vi "Build ATM Message.vi"(0 "Message Name":string, 5 "First Name":string, 7 "Last Name":string, 9 "Amount":dbl, 11 "error in":errorcluster) -> (4 "Message":string, 15 "error out":errorcluster)   [LabVIEW 2026, in "ATM.lvlib"]
doc: "Returns the ATM Messages text for a message name, multi-line as in the specification: Welcome, Main Menu (with First Name and Last Name), Verification Failed, Session Terminated, Deposit, Deposit Complete and Withdrawal Complete (with Amount, no decimals when whole), Withdrawal, Withdrawal Failed, Balance Inquiry (the balance on Amount, two decimals). An unknown name returns an empty string. An incoming error passes through."
uses:
  ATM.lvlib
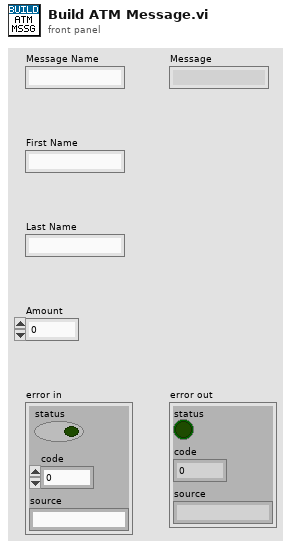
[diagram p1: front panel]
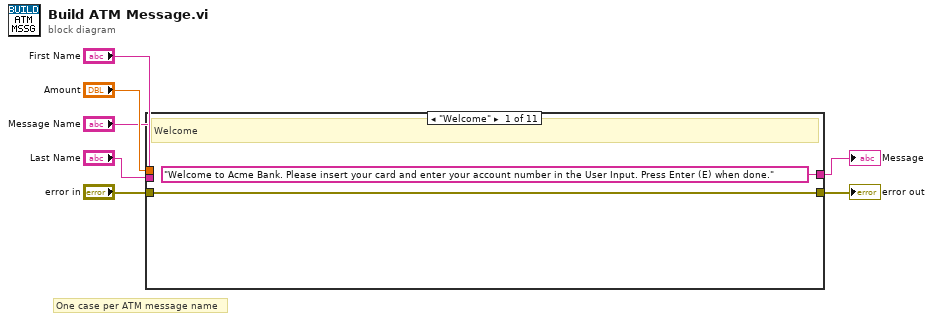
[diagram p0: block diagram]
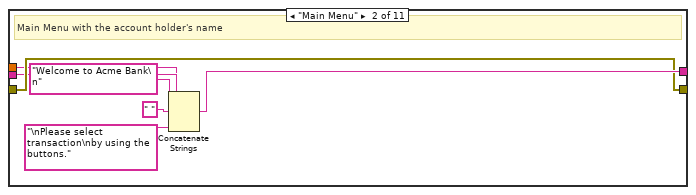
[diagram p2: hidden frame]
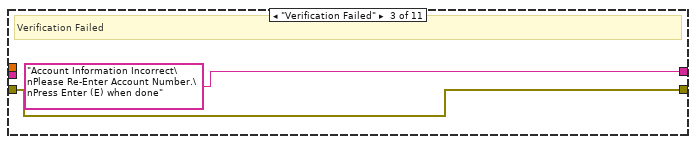
[diagram p3: hidden frame]
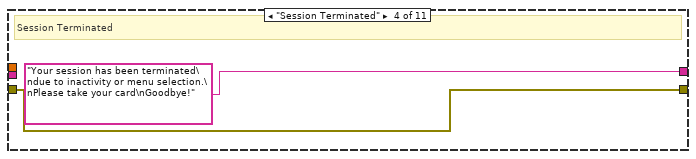
[diagram p4: hidden frame]
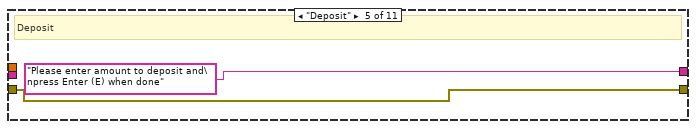
[diagram p5: hidden frame]
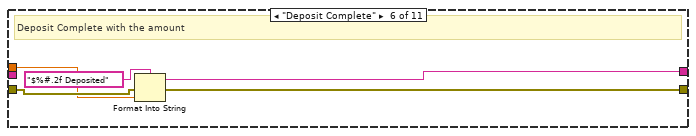
[diagram p6: hidden frame]
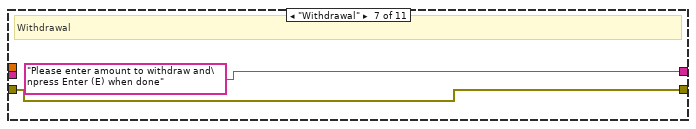
[diagram p7: hidden frame]
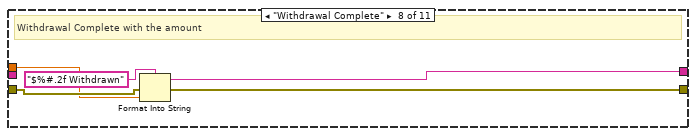
[diagram p8: hidden frame]
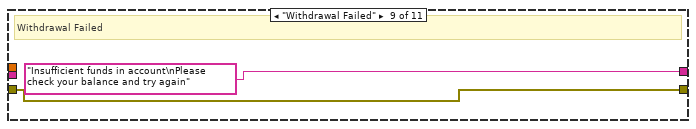
[diagram p9: hidden frame]
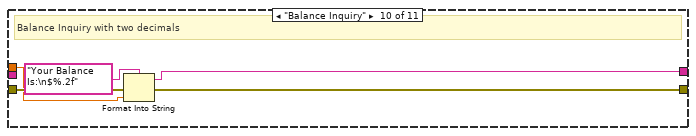
[diagram p10: hidden frame]
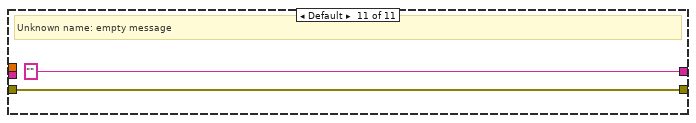
[diagram p11: hidden frame]
diagram:
  # "One case per ATM message name"
  n1 = case shown="\"Welcome\"" "Message Name" {
    tunnel: "First Name" -> [_ w10 _ _ _ _ _ _ _ _ _]
    tunnel: "Last Name" -> [_ w11 _ _ _ _ _ _ _ _ _]
    tunnel: "Amount" -> [_ _ _ _ _ w23 _ w30 _ w37 _]
    tunnel: "error in" -> [w8 w12 w17 w19 w21 w24 w28 w31 w35 w38 w42]
    tunnel: ["Welcome to Acme Bank. Please insert your card and enter your account number in the User Input. Press Enter (E) when done." ("Welcome text") w16 "Account Information Incorrect\nPlease Re-Enter Account Number.\nPress Enter (E) when done" ("Verification Failed text") "Your session has been terminated\ndue to inactivity or menu selection.\nPlease take your card\nGoodbye!" ("Session Terminated text") "Please enter amount to deposit and\npress Enter (E) when done" ("Deposit text") w26 "Please enter amount to withdraw and\npress Enter (E) when done" ("Withdrawal text") w33 "Insufficient funds in account\nPlease check your balance and try again" ("Withdrawal Failed text") w40 "" ("empty message")] -> w6
    tunnel: [w8 w12 w17 w19 w21 w27 w28 w34 w35 w41 w42] -> w7
    frame "Welcome" {
      # "Welcome"
    }
    frame "Main Menu" {
      # "Main Menu with the account holder's name"
      n2 = Concatenate Strings("Welcome to Acme Bank\n" ("Main Menu head"), w10, " " ("space"), w11, "\nPlease select transaction\nby using the buttons." ("Main Menu tail")) -> (w16:string)
    }
    frame "Verification Failed" {
      # "Verification Failed"
    }
    frame "Session Terminated" {
      # "Session Terminated"
    }
    frame "Deposit" {
      # "Deposit"
    }
    frame "Deposit Complete" {
      # "Deposit Complete with the amount"
      n3 = Format Into String(format string="$%#.2f Deposited", error in=w24, w23) -> (resulting string=w26:string, error out=w27:errorcluster)  [unwired: 1 in]
    }
    frame "Withdrawal" {
      # "Withdrawal"
    }
    frame "Withdrawal Complete" {
      # "Withdrawal Complete with the amount"
      n4 = Format Into String(format string="$%#.2f Withdrawn", error in=w31, w30) -> (resulting string=w33:string, error out=w34:errorcluster)  [unwired: 1 in]
    }
    frame "Withdrawal Failed" {
      # "Withdrawal Failed"
    }
    frame "Balance Inquiry" {
      # "Balance Inquiry with two decimals"
      n5 = Format Into String(format string="Your Balance Is:\n$%.2f", error in=w38, w37) -> (resulting string=w40:string, error out=w41:errorcluster)  [unwired: 1 in]
    }
    frame Default {
      # "Unknown name: empty message"
    }
  }
  "Message" <- w6
  "error out" <- w7
